vi "mail Message loop.vi"(8 "error in (no error)":errorcluster, 11 "Message Queues":T1) -> (0 "error out":errorcluster)   [LabVIEW 2026, in "Mail.lvlib"]
doc: "The message loop subVI to handle messages pertaining to logging data."
uses:
  support/Message Queue/All Message Queues.ctl
  support/Message Queue/Message Cluster.ctl
  Logging/Logging Configuration.ctl
  Logging/Logging State.ctl
  support/Message Queue/Enqueue Message (Single).vi
  <vilib>/Utility/error.llb/Error Cluster From Error Code.vi
  <vilib>/ErrorRing/Error Ring.xnode
  Mail.lvlib
  Logging/Logging.lvlib
  support/Message Queue/Message Queue.lvlib
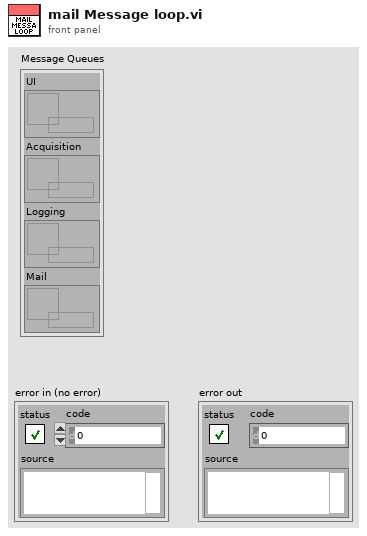
[diagram p1: front panel]
types:
  T1 = typedef "Message Queue.lvlib/All Message Queues.ctl" = cluster{"UI":refnum<queue>, "Acquisition":refnum<queue>, "Logging":refnum<queue>, "Mail":refnum<queue>}
  T2 = typedef "Logging.lvlib/Logging Configuration.ctl" = cluster{"Log File Base Path":path, "TDMS File Reference":refnum<k34>}
  T3 = typedef "Logging.lvlib/Logging State.ctl" = enum16{"Idle", "Logging"}
  T4 = enum16{"open", "open or create", "create or replace", "create", "open (read-only)"}
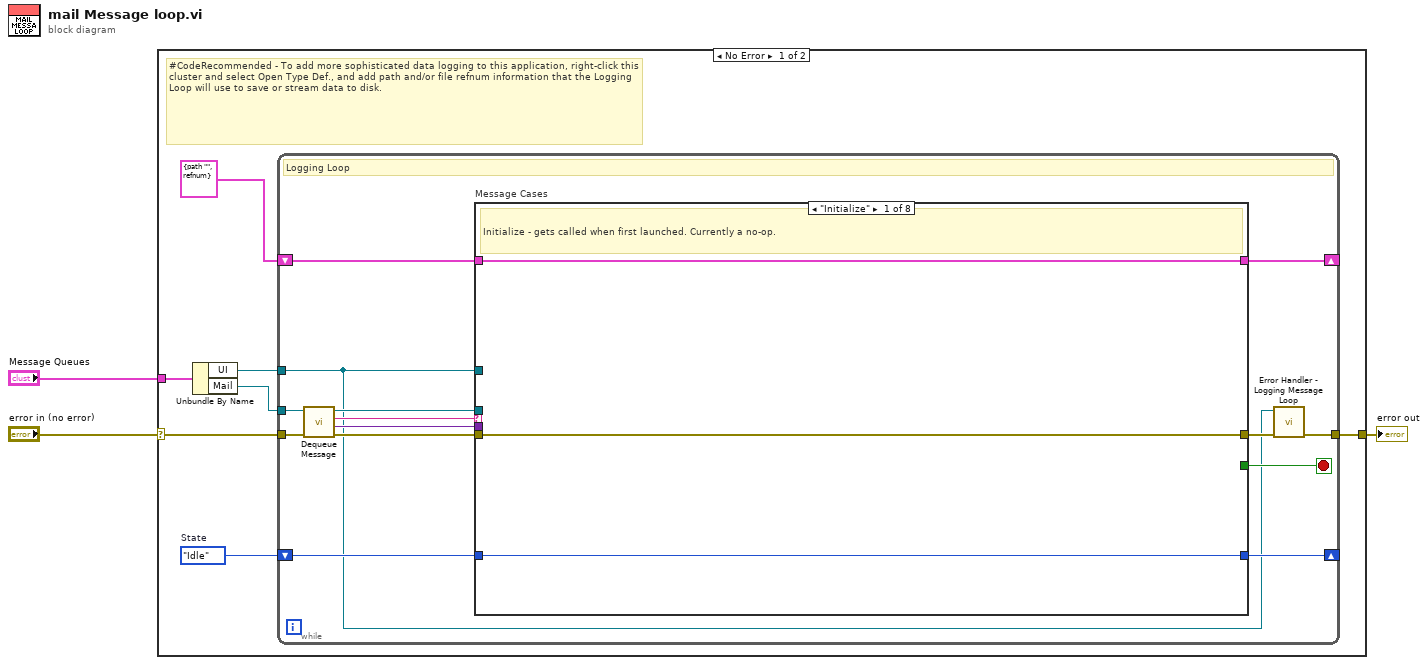
[diagram p0: block diagram]
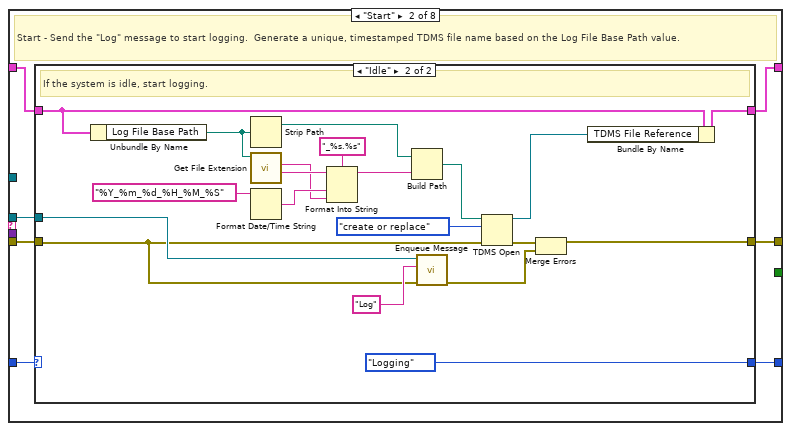
[diagram p2: hidden frame]
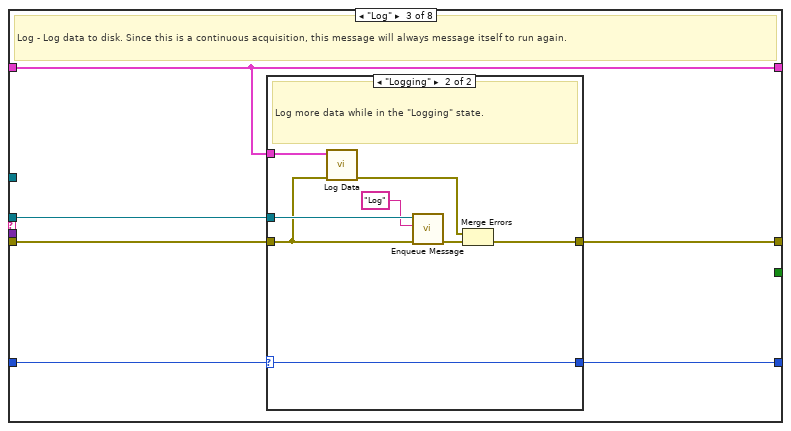
[diagram p4: hidden frame]
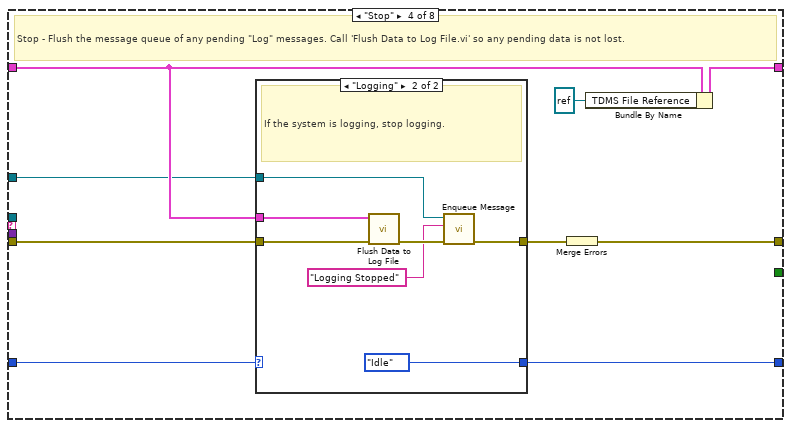
[diagram p6: hidden frame]
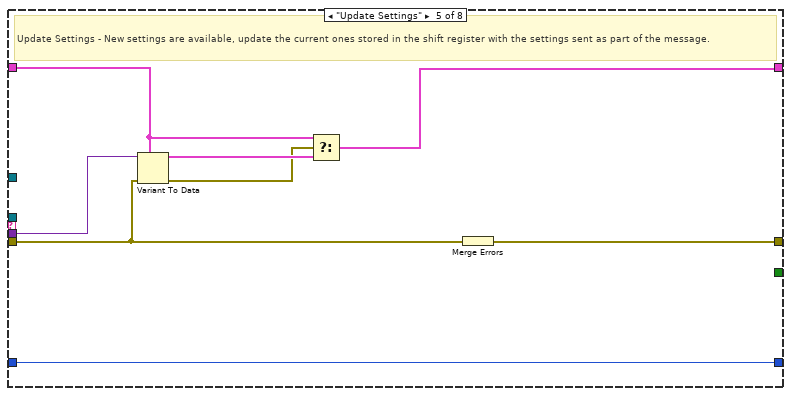
[diagram p8: hidden frame]
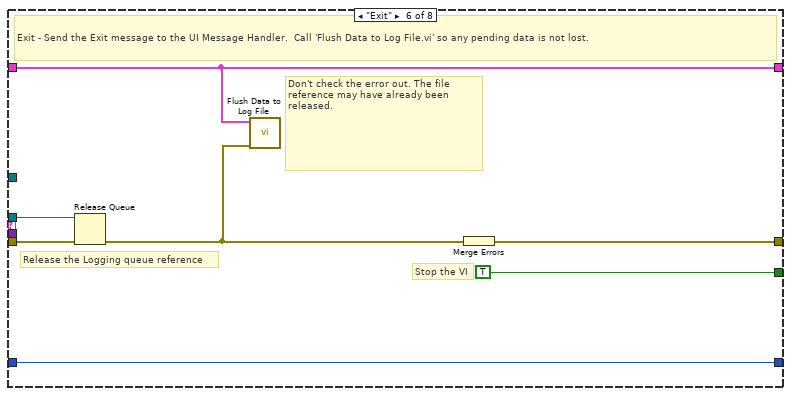
[diagram p9: hidden frame]
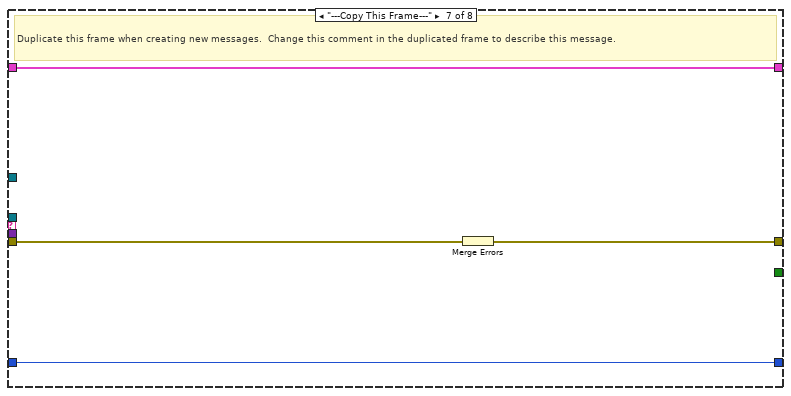
[diagram p10: hidden frame]
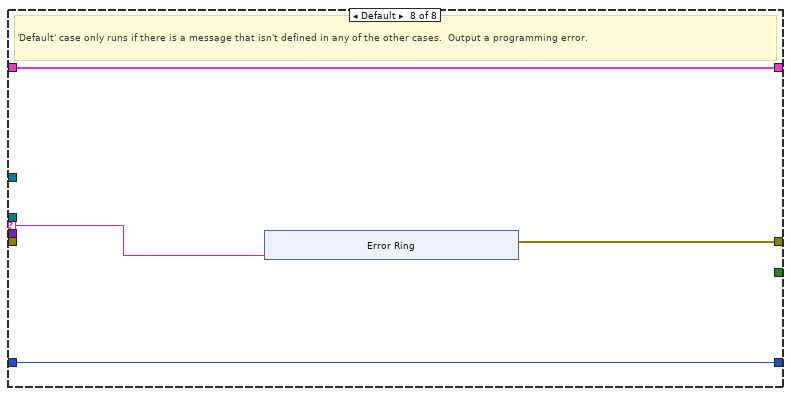
[diagram p11: hidden frame]
diagram:
  n1 = case shown="No Error" "error in (no error)" {
    selector: "error in (no error)" -> [w6 w122]
    tunnel: "Message Queues" -> [w10 _]
    tunnel: [w8 w122] -> w2
    frame No Error {
      w4 = Logging_State."Idle"  # State
      # "#CodeRecommended - To add more sophisticated data logging to this application, right-click this cluster and select Open Type Def., and add path and/or file refnum information that the Logging Loop will use to save or stream data to disk."
      n2 = Unbundle By Name(w10) -> ("UI"=w5:refnum<queue>, "Mail"=w9:refnum<queue>)
      n3 = while {
        tunnel: w9 -> [w16]
        shift-right: [w23] -> _
        shift-left: T2 {"Log File Base Path"=path "", "TDMS File Reference"=refnum} ("Logging Configuration") -> [w24]
        tunnel: w5 -> [w11]
        shift-right: [w14] -> _
        shift-left: w4 -> [w15]
        tunnel: w6 -> [w21]
        tunnel: [w13] -> w8
        stop <- w22 stop-if-true
        # "Logging Loop"
        n4 = call "Dequeue Message.vi"("error in (no error)"=w21, "Message Queue"=w16) -> ("error out"=w20:errorcluster, "Message Data"=w18:variant, "Message"=w19:string, "dup Message Queue"=w17:refnum<queue>)  [unwired: 6 in]
        n5 = case "Message Cases" shown="\"Initialize\"" w19 {
          selector: w19 -> [_ _ _ _ _ _ _ w111]
          tunnel: w17 -> [_ w33 w62 _ _ w103 _ _]
          tunnel: w20 -> [w26 w32 w61 w77 w93 w104 w110 _]
          tunnel: [w26 w34 w63 w82 w99 w105 w108 w112] -> w12
          tunnel: w24 -> [w27 w31 w60 w78 w97 w101 w109 w114]
          tunnel: [w27 w30 w60 w80 w94 w101 w109 w114] -> w23
          tunnel: [_ _ _ _ _ TRUE _ _] -> w22
          tunnel: w18 -> [_ _ _ _ w98 _ _ _]
          tunnel: w11 -> [_ _ _ w74 _ _ _ _]
          tunnel: w15 -> [w25 w29 w59 w76 w92 w100 w107 w113]
          tunnel: [w25 w28 w58 w75 w92 w100 w107 w113] -> w14
          frame "Initialize" {
            # "Initialize - gets called when first launched. Currently a no-op."
          }
          frame "Start" {
            # "Start - Send the \"Log\" message to start logging.  Generate a unique, timestamped TDMS file name based on the Log File Base Path value."
            n6 = case shown="\"Idle\"" w29 {
              selector: w29 -> [w36 _]
              tunnel: [w35 w39] -> w34
              tunnel: w33 -> [_ w40]
              tunnel: w32 -> [w35 w38]
              tunnel: w31 -> [w37 w41]
              tunnel: [w37 w43] -> w30
              tunnel: [w36 Logging_State."Logging" ("State")] -> w28
              frame "Logging" {
                # "The system is already logging. Ignore the \"Start\" message."
              }
              frame "Idle" {
                # "If the system is idle, start logging."
                n7 = Unbundle By Name(w41) -> ("Log File Base Path"=w56:path)
                n8 = Strip Path(path=w56) -> (stripped path=w53:path)  [unwired: 1 out]
                n9 = call <vilib>:"Get File Extension.vi"("file"=w56) -> ("filename without extension"=w54:string, "lowercase file extension"=w50:string)  [unwired: 6 in, 3 out]
                n10 = Format Date/Time String(time format string (%c)="%Y_%m_%d_%H_%M_%S") -> (date/time string=w51:string)  [unwired: 2 in]
                n11 = Format Into String(format string="_%s.%s", initial string=w54, w51, w50) -> (resulting string=w49:string)  [unwired: 1 in, 1 out]
                n12 = Build Path(base path=w53, name or relative path=w49) -> (appended path=w48:path)
                n13 = call-poly "Enqueue Message.vi"("error in (no error)"=w38, "Message"="Log", "Message Queue"=w40) -> ("error out"=w46:errorcluster)  [unwired: 7 in, 1 out]
                n14 = TDMS Open(8:w38, 10:T4."create or replace" ("operation (0:open)"), 11:w48) -> (0:w47:errorcluster, 3:w44:refnum<k34>)  [unwired: 4 in]
                n15 = Merge Errors(w47, w46) -> (w39:errorcluster)
                n16 = Bundle By Name(cluster=w41, "TDMS File Reference"=w44) -> (w43:T2)
              }
            }
          }
          frame "Log" {
            # "Log - Log data to disk. Since this is a continuous acquisition, this message will always message itself to run again."
            n17 = case shown="\"Logging\"" w59 {
              selector: w59 -> [w65 w67]
              tunnel: [w64 w73] -> w63
              tunnel: w62 -> [_ w71]
              tunnel: w61 -> [w64 w66]
              tunnel: w60 -> [_ w68]
              tunnel: [w65 w67] -> w58
              frame "Idle" {
                # "Ignore \"Log\" messages when the logging is idle."
              }
              frame "Logging" {
                # "Log more data while in the \"Logging\" state."
                n18 = call "Log Data.vi"("error in (no error)"=w66, "Logging Configuration"=w68) -> ("error out"=w70:errorcluster)  [unwired: 9 in]
                n19 = call-poly "Enqueue Message.vi"("error in (no error)"=w66, "Message"="Log", "Message Queue"=w71) -> ("error out"=w72:errorcluster)  [unwired: 7 in, 1 out]
                n20 = Merge Errors(w70, w72) -> (w73:errorcluster)
              }
            }
          }
          frame "Stop" {
            # "Stop - Flush the message queue of any pending \"Log\" messages. Call 'Flush Data to Log File.vi' so any pending data is not lost."
            n21 = case shown="\"Logging\"" w76 {
              selector: w76 -> [w83 _]
              tunnel: [w84 w87] -> w81
              tunnel: w78 -> [_ w90]
              tunnel: w77 -> [w84 w89]
              tunnel: [w83 Logging_State."Idle" ("State")] -> w75
              tunnel: w74 -> [_ w86]
              frame "Idle" {
                # "The system is already idle. Ignore the \"Stop\" message."
              }
              frame "Logging" {
                # "If the system is logging, stop logging."
                n22 = call "Flush Data to Log File.vi"("error in (no error)"=w89, "Logging Configuration"=w90) -> ("error out"=w91:errorcluster)  [unwired: 9 in]
                n23 = call-poly "Enqueue Message.vi"("error in (no error)"=w91, "Message"="Logging Stopped", "Message Queue"=w86) -> ("error out"=w87:errorcluster)  [unwired: 7 in, 1 out]
              }
            }
            n24 = Merge Errors(w81) -> (w82:errorcluster)
            n25 = Bundle By Name(cluster=w78, "TDMS File Reference"=refnum<k34> refnum) -> (w80:T2)
          }
          frame "Update Settings" {
            # "Update Settings - New settings are available, update the current ones stored in the shift register with the settings sent as part of the message."
            n26 = Variant To Data(error in=w93, type=w97, Variant=w98) -> (data=w96:T2, error out=w95:errorcluster)
            n27 = Select(t=w97, s=w95, f=w96) -> (s? t:f=w94:T2)
            n28 = Merge Errors(w93) -> (w99:errorcluster)
          }
          frame "Exit" {
            # "Don't check the error out. The file reference may have already been released."
            # "Release the Logging queue reference"
            # "Stop the VI"
            # "Exit - Send the Exit message to the UI Message Handler.  Call 'Flush Data to Log File.vi' so any pending data is not lost."
            n29 = Release Queue(queue=w103, error in (no error)=w104) -> (error out=w102:errorcluster)  [unwired: 1 in, 2 out]
            n30 = call "Flush Data to Log File.vi"("error in (no error)"=w102, "Logging Configuration"=w101) -> ()  [unwired: 9 in, 1 out]
            n31 = Merge Errors(w102) -> (w105:errorcluster)
          }
          frame "---Copy This Frame---" {
            # "Duplicate this frame when creating new messages.  Change this comment in the duplicated frame to describe this message."
            n32 = Merge Errors(w110) -> (w108:errorcluster)
          }
          frame Default {
            # "'Default' case only runs if there is a message that isn't defined in any of the other cases.  Output a programming error."
            n33 = xnode "Error Ring"("parameter 0"=w111) -> ("error out"=w112:errorcluster)
          }
        }
        n34 = call "Error Handler - Logging Message Loop.vi"("error in (no error)"=w12, "Message Queue"=w11) -> ("dup error in"=w13:errorcluster)  [unwired: 8 in, 1 out]
      }
    }
    frame Error {
    }
  }
  "error out" <- w2
